vi "Get Task by ID.vi"(7 "Project Store in":refnum<class "Project Store.lvclass">, 8 "error in (no error)":errorcluster, 11 "ID":string) -> (0 "error out":errorcluster, 2 "found?":bool, 3 "Task":T1, 5 "Project Store out":refnum<class "Project Store.lvclass">)   [LabVIEW 2024, in "Project Store.lvclass"]
doc: "Looks up the task with the given ID in the in-memory model. found? is FALSE and the row is empty when no task has that ID.\n\nGenerated by: Claude"
uses:
  Project Store.lvclass
  Rows/Task.ctl
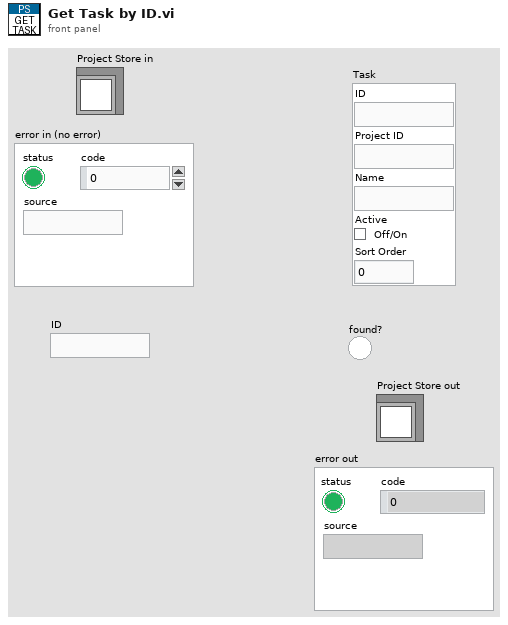
[diagram p1: front panel]
types:
  T1 = typedef "Task.ctl" = cluster{"ID":string, "Project ID":string, "Name":string, "Active":bool, "Sort Order":i32}
  T2 = typedef "Task List.ctl" = T1[]
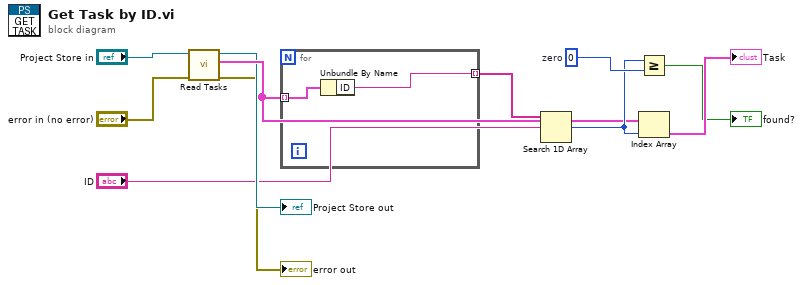
[diagram p0: block diagram]
diagram:
  w9 = 0  # zero
  n1 = call-dynamic "Read Tasks.vi"("error in (no error)"="error in (no error)", "Project Store in"="Project Store in") -> ("error out"=→"error out":errorcluster, "Task List"=w6:T2, "Project Store out"=→"Project Store out":refnum<class "Project Store.lvclass">)  [unwired: 7 in]
  n2 = for {
    tunnel: w6 -> [w12] mode=indexing
    tunnel: [w13] -> w7 mode=indexing
    n3 = Unbundle By Name(w12) -> ("ID"=w13:string)
  }
  n4 = Search 1D Array(1D array=w7, element="ID") -> (index of element=w8:i32)  [unwired: 1 in]
  n5 = Greater Or Equal?(x=w8, y=w9) -> (x >= y?=→"found?":bool)
  n6 = Index Array(array=w6, index=w8) -> (element=→"Task":T1)
